vi "Whitelist File Name--constant.vi"() -> (3 "Whitelist File Name":string)   [LabVIEW 2026]
doc: "Name of Hash Whitelist constant."
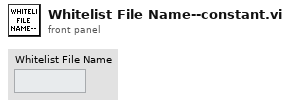
[diagram p1: front panel]
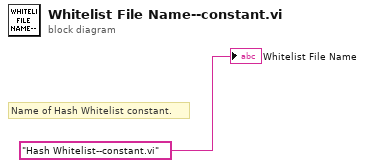
[diagram p0: block diagram]
diagram:
  # "Name of Hash Whitelist constant."
  "Whitelist File Name" <- "Hash Whitelist--constant.vi" ("Whitelist File Name")
